vi "FuncVI-FileSave.vi"(5 "InstanceRef":T2, 9 "arg list":T1[](array[typedef]) {"num" format="%.2f"}) -> (0 "error out":bool, 3 "result":T1 {"num" format="%.2f"})   [LabVIEW 2021]
doc: "::: CalcExpress Toolkit :::\nCopyright (c) 2000-2026 Konstantin Shifershteyn. All rights reserved."
uses:
  cetypes.llb/CalcExpress Function Argument Info.ctl
  cetypes.llb/CalcExpress Instance RefNum.ctl
panel:
  in  "max arg num":i32=3
  in  "min arg num":i32=3
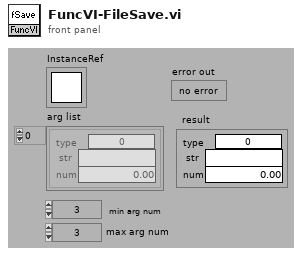
[diagram p1: front panel]
types:
  T1 = typedef "CalcExpress Function Argument Info.ctl" = cluster{"type":u32, "str":string, "num":dbl}
  T2 = typedef "CalcExpress Instance RefNum.ctl" = refnum<k1>
  T3 = enum32{"String", "DBL Number", "identifier", "1D Array of DBL", "2D Array of DBL", "CDB Number", "1D Array of CDB", "2D Array of CDB", "1D Array of String", "2D Array of String", "Unknown data type"}
  T4 = cluster{"index":i32, "data type":enum32{"String", "DBL Number", "identifier", "1D Array of DBL", "2D Array of DBL", "CDB Number", "1D Array of CDB", "2D Array of CDB", "1D Array of String", "2D Array of String", "Unknown data type"}, "default num":dbl, "default str":string}[]
  T5 = cluster{"function (open:0)":enum16{"open", "open or create", "create or replace", "create"}, "pos mode (0:2)":enum16{"start", "end", "current"}, "select mode (2)":enum32{"existing file", "new file", "new or existing file", "existing dir", "new dir", "new or existing dir", "existing file (use LLBs)", "new file (use LLBs)", "new or existing file (use LLBs)", "new or existing file or directory (use LLBs)", "existing dir (use LLBs)", "new dir (use LLBs)", "new or existing dir (use LLBs)", "existing file or dir", "new file or dir", "new or existing file or dir", "existing file or dir (use LLBs)", "new file or dir (use LLBs)"}}[]
  T6 = cluster{"function (open:0)":enum16{"open", "open or create", "create or replace", "create"}, "pos mode (0:2)":enum16{"start", "end", "current"}, "select mode (2)":enum32{"existing file", "new file", "new or existing file", "existing dir", "new dir", "new or existing dir", "existing file (use LLBs)", "new file (use LLBs)", "new or existing file (use LLBs)", "new or existing file or directory (use LLBs)", "existing dir (use LLBs)", "new dir (use LLBs)", "new or existing dir (use LLBs)", "existing file or dir", "new file or dir", "new or existing file or dir", "existing file or dir (use LLBs)", "new file or dir (use LLBs)"}}
  T7 = enum16{"open", "open or create", "create or replace", "create"}
  T8 = enum32{"existing file", "new file", "new or existing file", "existing dir", "new dir", "new or existing dir", "existing file (use LLBs)", "new file (use LLBs)", "new or existing file (use LLBs)", "new or existing file or directory (use LLBs)", "existing dir (use LLBs)", "new dir (use LLBs)", "new or existing dir (use LLBs)", "existing file or dir", "new file or dir", "new or existing file or dir", "existing file or dir (use LLBs)", "new file or dir (use LLBs)"}
  T9 = cluster{"type: use this constant to specify a predefined type code":enum32{"String", "DBL Number", "identifier", "1D Array of DBL", "2D Array of DBL", "CDB Number", "1D Array of CDB", "2D Array of CDB", "1D Array of String", "2D Array of String", "Unknown data type"}, string, "code":dbl}
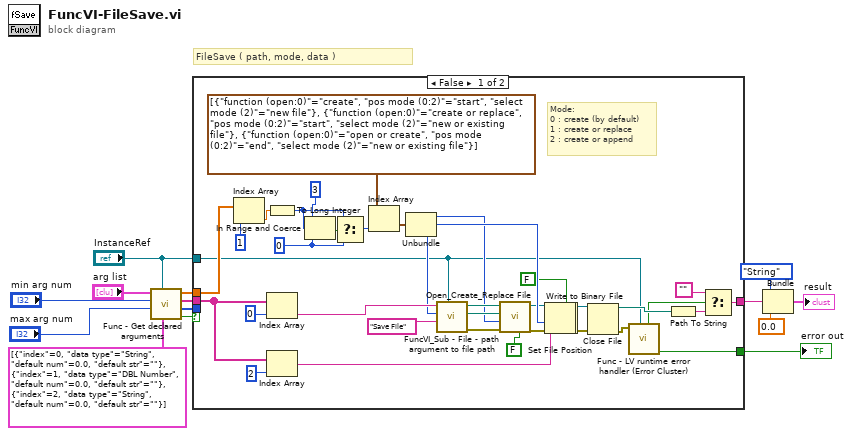
[diagram p0: block diagram]
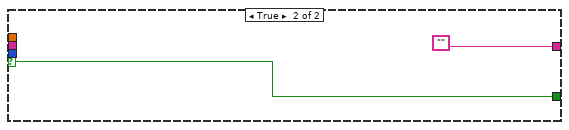
[diagram p2: hidden frame]
diagram:
  # "FileSave ( path, mode, data )"
  n1 = call "Func - Get declared arguments.vi"("arg descriptors"=T4 [{"index"=0, "data type"=enum."String", "default num"=0.0, "default str"=""}, {"index"=1, "data type"=enum."DBL Number", "default num"=0.0, "default str"=""}, {"index"=2, "data type"=enum."String", "default num"=0.0, "default str"=""}] ("args descriptors"), "InstanceRef"="InstanceRef", "max arg num"="max arg num", "min arg num"="min arg num", "arg list"="arg list") -> ("error out"=w10:bool, "type list"=w8:u32[], "str list"=w11:string[], "num list"=w9:dbl[])  [unwired: 3 in]
  n2 = case shown="False" w10 {
    selector: w10 -> [_ w54]
    tunnel: [w18 w54] -> w14
    tunnel: "InstanceRef" -> [w19 _]
    tunnel: w11 -> [w32 _]
    tunnel: w9 -> [w33 _]
    tunnel: w8 -> [_ _]
    tunnel: [w22 ""] -> w3
    frame False {
      w43 = 0 ("lo")
      # "Mode:\n0 : create (by default)\n1 : create or replace\n2 : create or append"
      n3 = Index Array(array=w33, index=1) -> (element=w47:dbl)
      n4 = To Long Integer(number=w47) -> (32bit integer=w41:i32)
      n5 = Index Array(array=w32, index=0) -> (element=w50:string)
      n6 = Index Array(array=w32, index=2) -> (element=w26:string)
      n7 = In Range and Coerce(upper limit=3 ("hi"), x=w41, lower limit=w43) -> (In Range?=w44:bool)  [unwired: 1 out]
      n8 = Select(t=w41, s=w44, f=w43) -> (s? t:f=w40:i32)
      n9 = Index Array(array=T5 [{"function (open:0)"=enum."create", "pos mode (0:2)"=enum."start", "select mode (2)"=enum."new file"}, {"function (open:0)"=enum."create or replace", "pos mode (0:2)"=enum."start", "select mode (2)"=enum."new or existing file"}, {"function (open:0)"=enum."open or create", "pos mode (0:2)"=enum."end", "select mode (2)"=enum."new or existing file"}], index=w40) -> (element=w45:T6)
      n10 = Unbundle(w45) -> ("function (open:0)"=w38:T7, "pos mode (0:2)"=w39:enum16{"start", "end", "current"}, "select mode (2)"=w35:T8)
      n11 = call "FuncVI_Sub - File - path argument to file path.vi"("InstanceRef"=w19, "prompt"="Save File", "select mode (2)"=w35, "arg: file path"=w50) -> ("error out"=w37:errorcluster, "base path"=w49:path, "file path"=w52:path)  [unwired: 5 in]
      n12 = call <vilib>:"Open_Create_Replace File.vi"("advisory dialog? (display:T)"=FALSE, "error in (no error)"=w37, "function (open:0)"=w38, "start path  (Not A Path)"=w49, "file path"=w52) -> ("error out"=w30:errorcluster, "refnum"=w31:refnum<file>)  [unwired: 3 in, 2 out]
      n13 = Set File Position(refnum=w31, from (0:start)=w39, error in=w30) -> (refnum out=w17:refnum<file>, error out=w16:errorcluster)  [unwired: 1 in]
      n14 = Write to Binary File(file (use dialog)=w17, data=w26, error in=w16, 5:FALSE ("prepend array or string size? (T)")) -> (refnum out=w29:refnum<file>, error out=w28:errorcluster)  [unwired: 2 in, 1 out]
      n15 = Close File(refnum=w29, error in=w28) -> (path=w25:path, error out=w21:errorcluster)
      n16 = call "Func - LV runtime error handler (Error Cluster).vi"("InstanceRef"=w19, "LabVIEW error"=w21) -> ("error out"=w18:bool, "LV error status"=w20:bool)  [unwired: 4 in, 2 out]
      n17 = Path To String(path=w25) -> (string=w24:string)
      n18 = Select(t="", s=w20, f=w24) -> (s? t:f=w22:string)
    }
    frame True {
    }
  }
  "error out" <- w14
  n19 = Bundle("type: use this constant to specify a predefined type code"=T3."String", w3, "code"=0.0) -> (→"result":T9)  [unwired: 1 in]
